vi "GenNewTraj.vi"(6 "Drive Type":T1, 7 "Turn Rate":dbl=5.0 format="%#_13g", 8 "Stoopid Overlap %":dbl min=0.0, 9 "Path Type":T6, 10 "Parameters":T5 {"Limits"."StoopidFast (fps)" min=0.0; "Limits"."Jerk (fps^3)" min=0.0 step=1.0; "Limits"."Accel (fps^2)" min=0.0; "Limits"."Velocity (fps)" min=0.0; "Overrides"."Angle Override" step=5.0; "Overrides"."Velocity Override" step=5.0; "Overrides"."Angular Override" step=5.0; "Angular Limits"."Jerk (deg/s^3)" min=0.0 step=1.0; "Angular Limits"."Accel (deg/s^2)" min=0.0; "Angular Limits"."Velocity (deg/s)" min=0.0}, 11 "Points in":cluster{"x":dbl, "y":dbl, "th":dbl}[](array[cluster])) -> (0 "Time & Dist":cluster{"Time (s)":dbl, "Distance (ft)":dbl}, 1 "Valid":bool, 2 "Trajectory Data":T7, 3 "Updated Waypoints":cluster{"x":dbl, "y":dbl, "th":dbl}[](array[cluster]))   [LabVIEW 2023]
uses:
  Types/Trajectory Data.ctl
  Types/Segment Type.ctl
  Types/Path Type.ctl
  Types/Limits.ctl
  Types/Overrides.ctl
  Types/Angluar Limits.ctl
  Types/Drive Type.ctl
  Bezier/Bezier Trajectory.vi
  Clothoid/Generate Clothoid Trajectory.vi
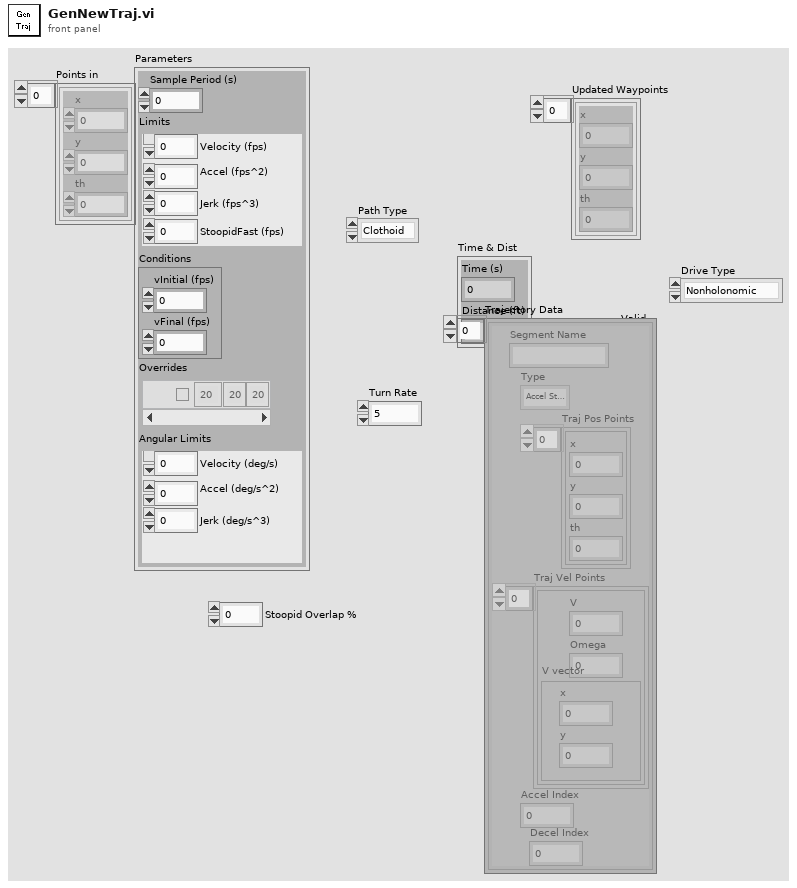
[diagram p1: front panel]
types:
  T1 = typedef "Drive Type.ctl" = enum16{"Nonholonomic", "Holonomic"}
  T2 = typedef "Limits.ctl" = cluster{"Velocity (fps)":dbl, "Accel (fps^2)":dbl, "Jerk (fps^3)":dbl, "StoopidFast (fps)":dbl}
  T3 = typedef "Overrides.ctl" = cluster{"Count":string, "Angular Override":dbl, "Enabled?":bool, "Velocity Override":dbl, "Angle Override":dbl}[]
  T4 = typedef "Angluar Limits.ctl" = cluster{"Velocity (deg/s)":dbl, "Accel (deg/s^2)":dbl, "Jerk (deg/s^3)":dbl}
  T5 = cluster{"Sample Period (s)":dbl, "Limits":T2, "Conditions":cluster{"vInitial (fps)":dbl, "vFinal (fps)":dbl}, "Overrides":T3, "Angular Limits":T4}
  T6 = typedef "Path Type.ctl" = enum16{"Clothoid", "Bezier"}
  T7 = typedef "Trajectory Data.ctl" = cluster{"Segment Name":string, "Type":T8, "Traj Pos Points":cluster{"x":dbl, "y":dbl, "th":dbl}[], "Traj Vel Points":cluster{"V":dbl, "Omega":dbl, "V vector":cluster{"y":dbl, "x":dbl}}[], "Accel Index":i32, "Decel Index":i32}[]
  T8 = typedef "Segment Type.ctl" = enum16{"Accel Straight", "Const Straight", "Blend", "Circle", "Bezier"}
  T9 = cluster{"vInitial (fps)":dbl, "vFinal (fps)":dbl}
  T10 = cluster{"Segment Name":string, "Type":T8, "Traj Pos Points":cluster{"x":dbl, "y":dbl, "th":dbl}[], "Traj Vel Points":cluster{"V":dbl, "Omega":dbl, "V vector":cluster{"y":dbl, "x":dbl}}[], "Accel Index":i32, "Decel Index":i32}[]
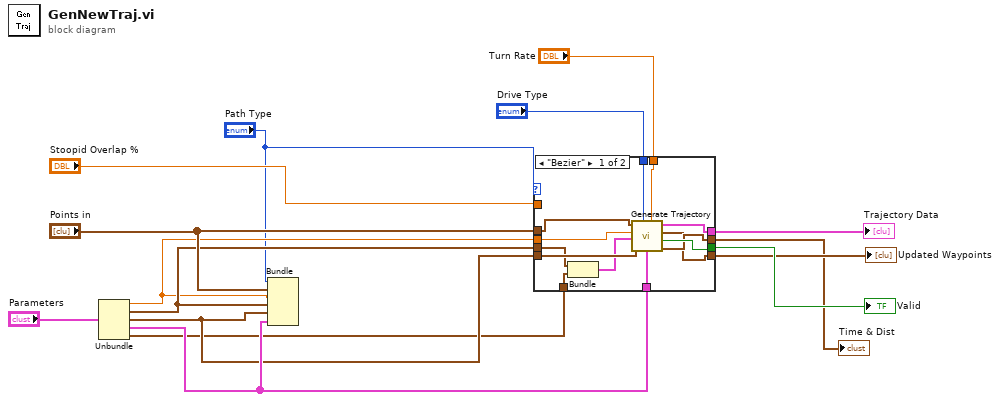
[diagram p0: block diagram]
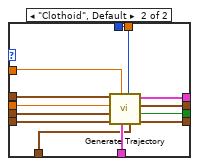
[diagram p2: hidden frame]
diagram:
  n1 = Unbundle("Parameters") -> ("Sample Period (s)"=w7:dbl, "Limits"=w10:T2, "Conditions"=w9:T9, "Overrides"=w12:T3, "Angular Limits"=w3:T4)
  n2 = Bundle("Path Type"="Path Type", "Points in"="Points in", "Sample Period (s)"=w7, "Limits"=w10, "Conditions"=w9, "Overrides"=w12) -> ()  [unwired: 1 in, 1 out]
  n3 = case shown="\"Bezier\"" "Path Type" {
    tunnel: [w25 w40] -> w15
    tunnel: [w23 w39] -> w8
    tunnel: w9 -> [w27 w38]
    tunnel: w10 -> [w19 w37]
    tunnel: w12 -> [w26 w36]
    tunnel: [w22 w35] -> w14
    tunnel: [w24 w30] -> w6
    tunnel: "Stoopid Overlap %" -> [_ w34]
    tunnel: "Points in" -> [w28 w33]
    tunnel: w7 -> [w21 w32]
    tunnel: "Drive Type" -> [w20 w31]
    tunnel: w3 -> [w18 w29]
    tunnel: "Turn Rate" -> [w16 _]
    frame "Bezier" {
      n4 = Bundle("Limits"=w19, "Angular Limits"=w18) -> (w17:cluster{"Limits":T2, "Angular Limits":T4})  [unwired: 1 in]
      n5 = call-poly "Generate Trajectory.vi"("Turn Rate"=w16, "Overrides"=w26, "Drive Type"=w20, "Conditions"=w27, "All Limits"=w17, "sample period (s)"=w21, "WayPoints"=w28) -> ("Time & Dist"=w23:cluster{"Time (s)":dbl, "Distance (ft)":dbl}, "Valid"=w25:bool, "Updated Waypoints"=w22:cluster{"x":dbl, "y":dbl, "th":dbl}[], "Trajectory Data"=w24:T7)  [unwired: 1 in]
    }
    frame "Clothoid", Default {
      n6 = call-poly "Generate Trajectory.vi"("Angular Limits"=w29, "Drive Type"=w31, "Overrides"=w36, "Stoopid Overlap %"=w34, "Conditions"=w38, "Limits"=w37, "Sample Period (s)"=w32, "WayPoints"=w33) -> ("Updated Waypoints"=w35:cluster{"x":dbl, "y":dbl, "th":dbl}[], "Valid"=w40:bool, "Time & Dist"=w39:cluster{"Time (s)":dbl, "Distance (ft)":dbl}, "Trajectory Data Out"=w30:T10)
    }
  }
  "Valid" <- w15
  "Updated Waypoints" <- w14
  "Time & Dist" <- w8
  "Trajectory Data" <- w6
